vi "Begin Undo.vi"(6 "Transaction Name":string, 8 "error in (no error)":errorcluster, 11 "Vi Ref":refnum<vi>) -> (0 "error out":errorcluster, 3 "Vi Ref Out":refnum<vi>)   [LabVIEW 2012, in "Scripting Tools.lvlib"]
doc: "Begins the Undo transaction for the referenced vi"
uses:
  Scripting Tools.lvlib
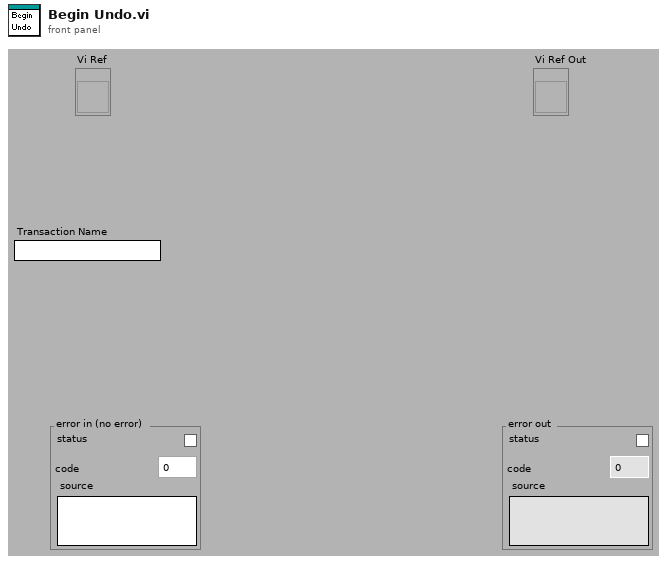
[diagram p1: front panel]
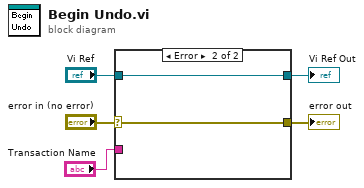
[diagram p0: block diagram]
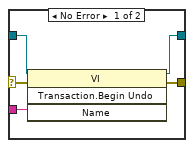
[diagram p2: hidden frame]
diagram:
  n1 = case shown="Error" "error in (no error)" {
    selector: "error in (no error)" -> [w10 w11]
    tunnel: [w9 w11] -> w4
    tunnel: "Vi Ref" -> [w8 w12]
    tunnel: [w7 w12] -> w2
    tunnel: "Transaction Name" -> [w6 _]
    frame No Error {
      n2 = invoke class="VI" method="Transaction.Begin Undo"(reference=w8, error in=w10, "Name"=w6) -> (reference out=w7:refnum<vi>, error out=w9:errorcluster)  [unwired: 1 in, 2 out]
    }
    frame Error {
    }
  }
  "error out" <- w4
  "Vi Ref Out" <- w2
